vi "Set Port.vi"(8 "error in (no error)":errorcluster caption="에러 입력(에러 없음)", 11 "CE RF Switch Box 입력":refnum<class "CE RF Switch Box.lvclass">) -> (0 "error out":errorcluster caption="에러 출력", 3 "CE RF Switch Box 출력":refnum<class "CE RF Switch Box.lvclass">)   [LabVIEW 2023, in "RF Switch Box.lvlib" / "CE RF Switch Box.lvclass"]
uses:
  CE RF Switch Box.lvclass
  CE RF Switch Box.lvclass/CE RF Switch Box.ctl
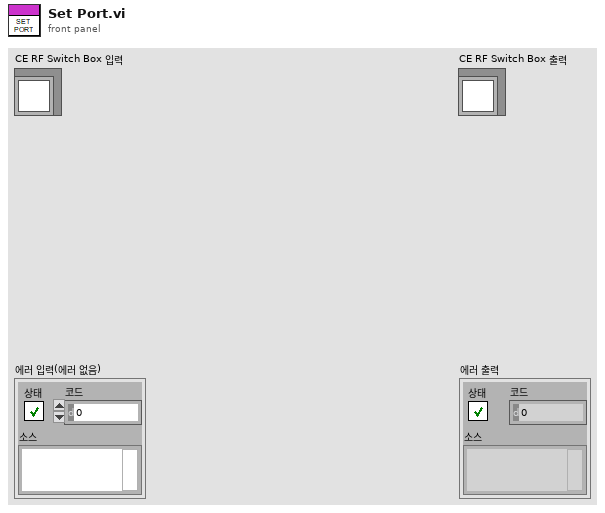
[diagram p1: front panel]
types:
  T1 = typedef "RF Switch Box.lvlib/Filter path.ctl" = enum16{"Thru", "Direct Amp", "1G HPF", "3G HPF", "7G HPF", "6G HPF", "port 1", "port 2", "port 3", "port 4", "port 5", "port 6", "port 7", "port 8", "port 9", "port 10", "port 11", "port 12", "port 13", "port 14", "port 15", "port 16", "port 17", "port 18"}
  T2 = typedef "RF Switch Box.lvlib/Input path.ctl" = enum16{"Input 1", "Input 2", "Input 3"}
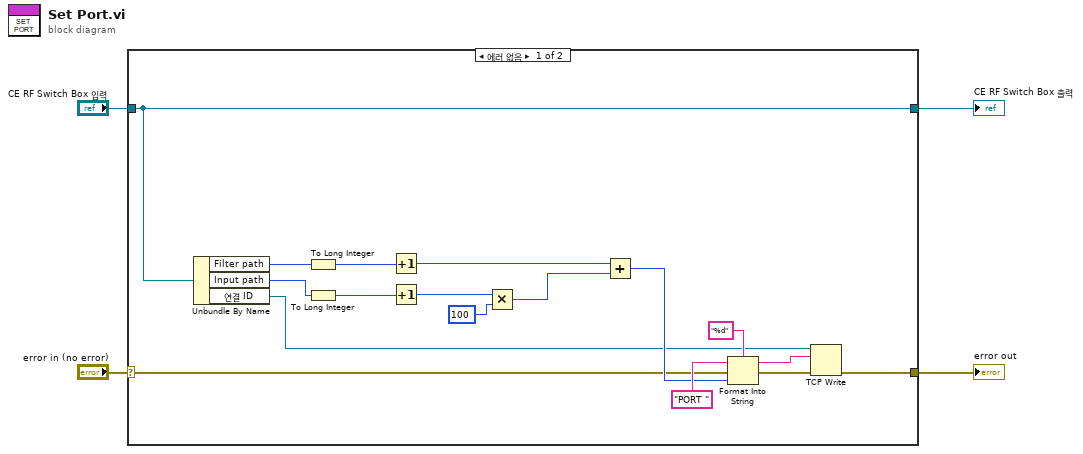
[diagram p0: block diagram]
diagram:
  n1 = case shown="에러 없음" "error in (no error)" {
    selector: "error in (no error)" -> [w8 w23]
    tunnel: [w6 w23] -> w3
    tunnel: [w10 w22] -> w1
    tunnel: "CE RF Switch Box 입력" -> [w10 w22]
    frame No Error {
      n2 = Unbundle By Name(w10) -> ("Filter path"=w18:T1, "Input path"=w21:T2, "연결 ID"=w9:refnum<k5>)
      n3 = To Long Integer(number=w18) -> (32bit integer=w19:i32)
      n4 = To Long Integer(number=w21) -> (32bit integer=w20:i32)
      n5 = Increment(x=w19) -> (x+1=w15:i32)
      n6 = Increment(x=w20) -> (x+1=w17:i32)
      n7 = Multiply(x=w17, y=100) -> (x*y=w14:i32)
      n8 = Add(x=w15, y=w14) -> (x+y=w11:i32)
      n9 = Format Into String(format string="%d" ("포맷 문자열"), initial string="PORT " ("초기 문자열"), error in=w8, w11) -> (resulting string=w5:string, error out=w7:errorcluster)
      n10 = TCP Write(connection ID=w9, data in=w5, error in (no error)=w7) -> (error out=w6:errorcluster)  [unwired: 1 in, 2 out]
    }
    frame Error {
    }
  }
  "error out" <- w3
  "CE RF Switch Box 출력" <- w1
